vi "trace.payload_received.vi"(8 "dataflow error in":errorcluster, 10 "Response":string="<empty string>", 11 "Path":string) -> (0 "dataflow error out":errorcluster)   [LabVIEW 2020, in "Nominal Client.lvclass"]
uses:
  Nominal Client.lvclass
  <vilib>/Utility/libraryn.llb/Get File Extension.vi
  Nominal Client.lvclass/Nominal Client.ctl
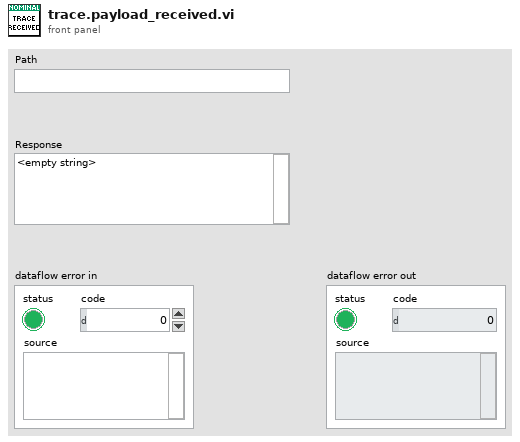
[diagram p1: front panel]
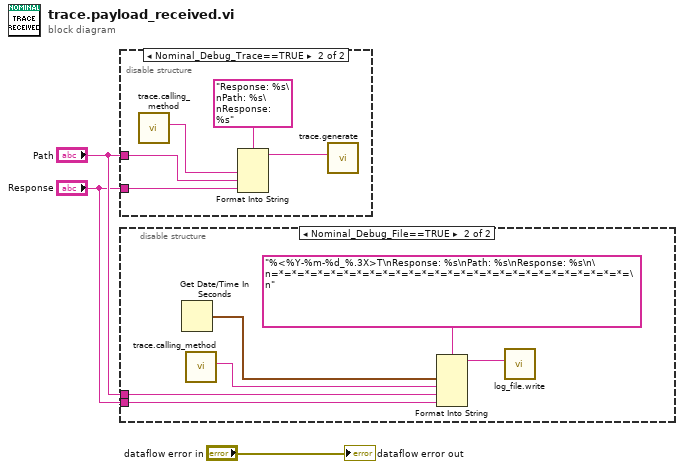
[diagram p0: block diagram]
diagram:
  n1 = disable-structure shown="Nominal_Debug_Trace==TRUE" {
    disable-tunnel: "Response" -> [_ w7]
    disable-tunnel: "Path" -> [_ w6]
    frame condition #0 {
    }
    frame condition #1 (active) {
      n2 = call "trace.calling_method.vi"() -> ("Calling Method Name"=w4:string)  [unwired: 11 in]
      n3 = Format Into String(format string="Response: %s\nPath: %s\nResponse: %s", w4, w6, w7) -> (resulting string=w8:string)  [unwired: 2 in, 1 out]
      n4 = call "trace.generate.vi"("trace string"=w8) -> ()  [unwired: 11 in]
    }
  }
  n5 = disable-structure shown="Nominal_Debug_File==TRUE" {
    disable-tunnel: "Response" -> [_ w14]
    disable-tunnel: "Path" -> [_ w13]
    frame condition #0 {
    }
    frame condition #1 (active) {
      n6 = Get Date/Time In Seconds() -> (seconds since 1Jan1904=w9:timestamp)
      n7 = call "trace.calling_method.vi"() -> ("Calling Method Name"=w11:string)  [unwired: 11 in]
      n8 = Format Into String(format string="%<%Y-%m-%d_%.3X>T\nResponse: %s\nPath: %s\nResponse: %s\n\n=*=*=*=*=*=*=*=*=*=*=*=*=*=*=*=*=*=*=*=*=*=*=*=*=*=*=*=\n", w9, w11, w13, w14) -> (resulting string=w10:string)  [unwired: 2 in, 1 out]
      n9 = call "log_file.write.vi"("trace string"=w10) -> ()  [unwired: 11 in]
    }
  }
  "dataflow error out" <- "dataflow error in"
